vi "Init DS and IO.vi"(8 "error in":errorcluster, 9 "Code ready":bool=TRUE, 11 "OpModes":T1) -> (0 "error out":errorcluster, 3 "OpModes":T1)   [LabVIEW 2023]
doc: "Update the DS and dashboards about opModes available for selection, initialize the robot controller I/O, and indicate whether robot code is ready to be run.\nIf your code has lots of computation before it is ready, you can pass false for Code Ready and make your own call to Set User Code Ready."
uses:
  <vilib>/MRC/MrcLib.lvlib
  <vilib>/Rock Robotics/Network Tables/NT Write String Array.vi
  <vilib>/MRC/MrcLib/VIs/Robot Framework/DS OpModes.ctl
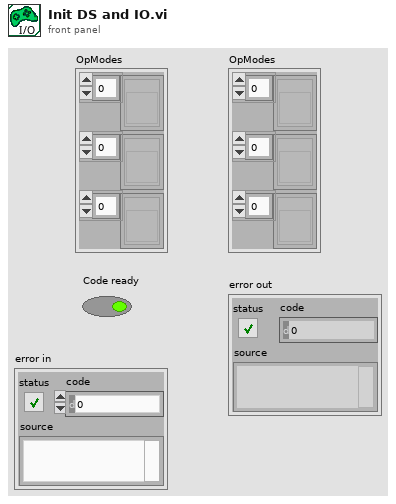
[diagram p1: front panel]
types:
  T1 = typedef "DS OpModes.ctl" = cluster{"Autos":refnum<vi>[], "Teles":refnum<vi>[], "Utilities":refnum<vi>[]}
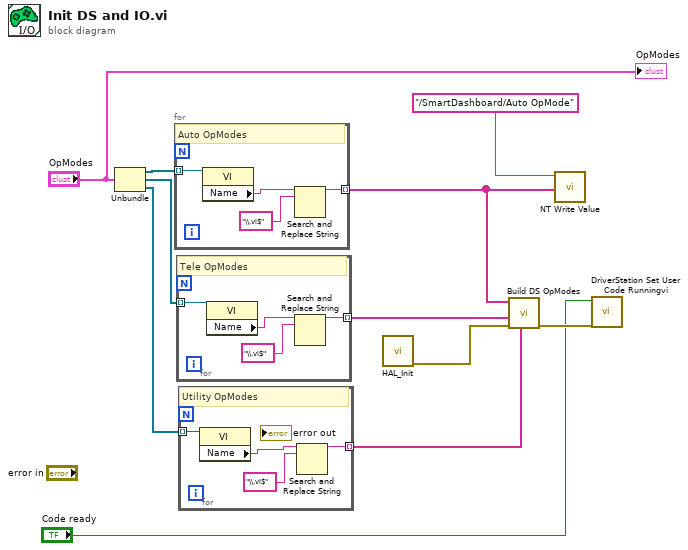
[diagram p0: block diagram]
diagram:
  n1 = Unbundle("OpModes") -> ("Autos"=w11:refnum<vi>[], "Teles"=w10:refnum<vi>[], "Utilities"=w8:refnum<vi>[])
  n2 = for {
    tunnel: w11 -> [w13] mode=indexing
    tunnel: [w14] -> w4 mode=indexing
    # "Auto OpModes"
    n3 = property class="VI"(reference=w13) -> ("Name"=w12:string)  [unwired: 1 in, 2 out]
    n4 = Search and Replace String(input string=w12, search string="\\.vi$") -> (result string=w14:string)  [unwired: 6 in, 3 out]
  }
  n5 = for {
    tunnel: w10 -> [w17] mode=indexing
    tunnel: [w18] -> w6 mode=indexing
    # "Tele OpModes"
    n6 = property class="VI"(reference=w17) -> ("Name"=w16:string)  [unwired: 1 in, 2 out]
    n7 = Search and Replace String(input string=w16, search string="\\.vi$") -> (result string=w18:string)  [unwired: 6 in, 3 out]
  }
  n8 = for {
    tunnel: w8 -> [w21] mode=indexing
    tunnel: [w22] -> w5 mode=indexing
    # "Utility OpModes"
    n9 = property class="VI"(reference=w21) -> ("Name"=w20:string)  [unwired: 1 in, 2 out]
    n10 = Search and Replace String(input string=w20, search string="\\.vi$") -> (result string=w22:string)  [unwired: 6 in, 3 out]
  }
  n11 = call <vilib>:"HAL_Init.vi"() -> ("error out"=w1:errorcluster)  [unwired: 11 in]
  n12 = call <vilib>:"Build DS OpModes.vi"("utility names"=w5, "error in (no error)"=w1, "tele names"=w6, "auto names"=w4) -> ("error in (no error) 2"=w3:errorcluster)  [unwired: 7 in]
  n13 = call-poly <vilib>:"NT Write Value.vi"("value"=w4, "name"="/SmartDashboard/Auto OpMode") -> ()  [unwired: 9 in, 1 out]
  n14 = call <vilib>:"DriverStation Set User Code Runningvi.vi"("error in (no error)"=w3, "code ready for enable"="Code ready") -> ()  [unwired: 9 in, 1 out]
  "OpModes" <- "OpModes"
